vi "Read JSON status.vi"(8 "error in (no error)":errorcluster, 11 "Camera in":refnum<class "Camera.lvclass">) -> (0 "error out":errorcluster, 2 "JSON status":T1, 3 "Camera out":refnum<class "Camera.lvclass">)   [LabVIEW 2018]
uses:
  Camera.lvclass
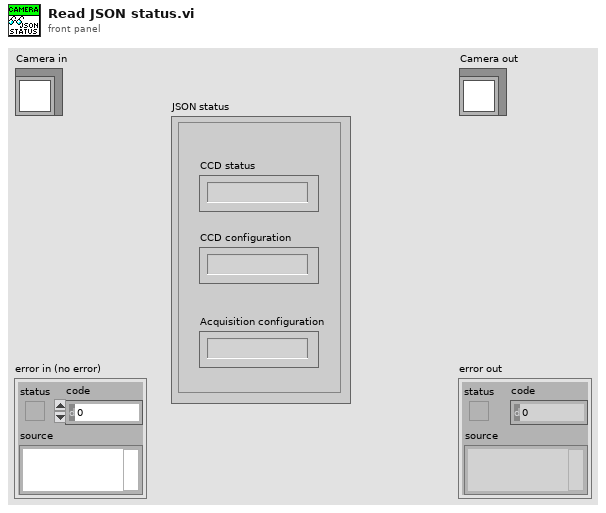
[diagram p1: front panel]
types:
  T1 = cluster{"CCD status":string, "CCD configuration":string, "Acquisition configuration":string}
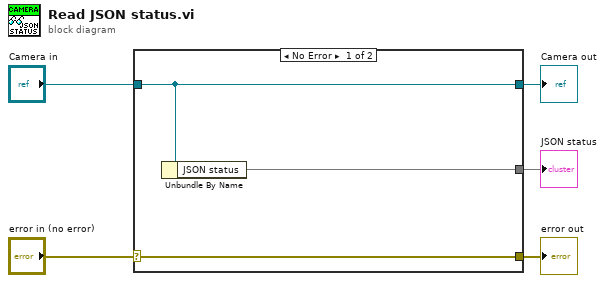
[diagram p0: block diagram]
diagram:
  n1 = case shown="No Error" "error in (no error)" {
    selector: "error in (no error)" -> [w8 w9]
    tunnel: [w8 w9] -> w4
    tunnel: [w7 w10] -> w2
    tunnel: "Camera in" -> [w7 w10]
    tunnel: [w6 _] -> w1
    frame No Error {
      n2 = Unbundle By Name(w7) -> ("JSON status"=w6)
    }
    frame Error {
    }
  }
  "error out" <- w4
  "Camera out" <- w2
  "JSON status" <- w1
